vi "Destroy Table Buffer.vi"(8 "error in":errorcluster, 11 "UI GUID":string) -> (0 "error out":errorcluster)   [LabVIEW 2025, in "CAN-LIN Raw Bus Capture UI.lvlib"]
uses:
  CAN-LIN Raw Bus Capture UI.lvlib
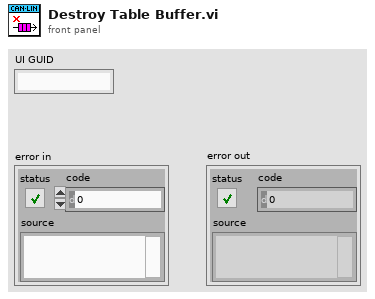
[diagram p1: front panel]
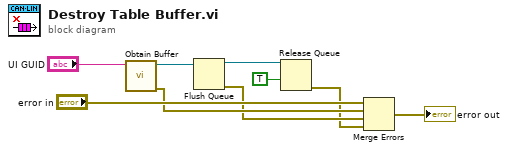
[diagram p0: block diagram]
diagram:
  n1 = call "Obtain Buffer.vi"("UI GUID"="UI GUID") -> ("error out"=w5:errorcluster, "Table Queue"=w7:refnum<queue>)  [unwired: 9 in]
  n2 = Flush Queue(queue=w7) -> (queue out=w6:refnum<queue>, error out=w4:errorcluster)  [unwired: 1 in, 1 out]
  n3 = Release Queue(queue=w6, force destroy? (F)=TRUE) -> (error out=w3:errorcluster)  [unwired: 1 in, 2 out]
  n4 = Merge Errors("error in", w5, w4, w3) -> (→"error out":errorcluster)
